vi "Get Service Class Instances.vi"(11 "GUID":string) -> (3 "service instances":refnum<class "ServiceBase.lvclass">[](array[class]))   [LabVIEW 2025, in "OOB gRPC Server.lvlib"]
uses:
  OOB gRPC Server.lvlib
  <vilib>/gRPC/LabVIEW gRPC Servicer/ServiceBase/ServiceBase.lvclass
  RPC Service/OOBgRPCService/OOBgRPCService.lvclass
  C:/Program Files/National Instruments/LabVIEW 2025/vi.lib/gRPC/LabVIEW gRPC Servicer/ServiceBase/ServiceBase.lvclass
  C:/Dev/measurement-plugin-automotive-interface-plugins/src/labview/can-lin/CAN-LIN Raw Bus Capture/OOB gRPC Server/RPC Service/OOBgRPCService/OOBgRPCService.lvclass
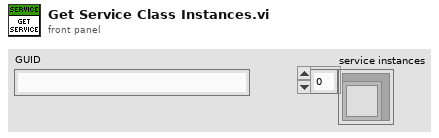
[diagram p1: front panel]
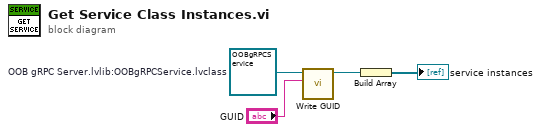
[diagram p0: block diagram]
diagram:
  w1 = refnum<class "OOBgRPCService.lvclass"> refnum  # OOB gRPC Server.lvlib:OOBgRPCService.lvclass
  n1 = call "Write GUID.vi"("GUID"="GUID", "OOBgRPCService in"=w1) -> ("OOBgRPCService out"=w2:refnum<class "OOBgRPCService.lvclass">)  [unwired: 8 in, 1 out]
  n2 = Build Array(w2) -> (→"service instances":refnum<class "OOBgRPCService.lvclass">[])
